vi "VIH HelpGen - Image - Fill Outer Regions in 2D Array.vi"(8 "New Color (transparent)":u32(colorbox)=16777216, 9 "Source Color (white)":u32=16777215 format="%.0x", 11 "Image Data in":u32[][](array[numeric]) format="%.0x") -> (3 "Image Data out":u32[][](array[numeric]) format="%.0x")   [LabVIEW 2014]
doc: "::: VI Helpeks :::\nCopyright (c) 2000-2026 Konstantin Shifershteyn. All rights reserved."
panel:
  out "Points replaces":i32
  out "Sub-regions found":i32
  # "VI Helpeks\nCopyright (c) 2012-2026 Konstantin Shifershteyn"
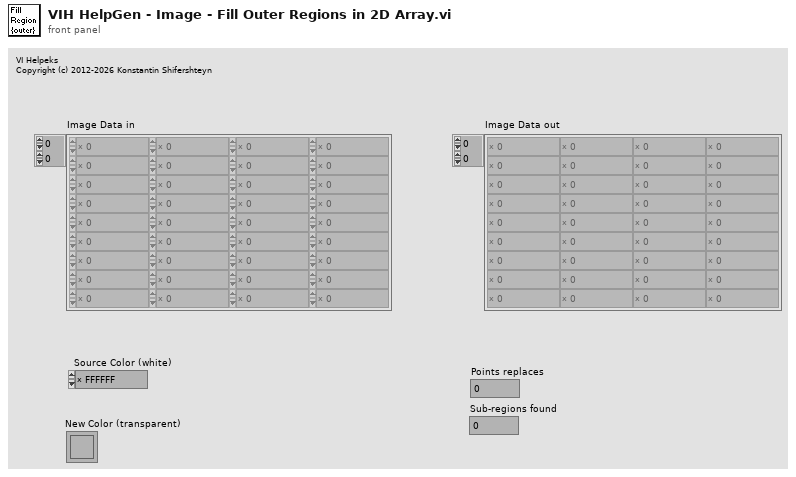
[diagram p1: front panel]
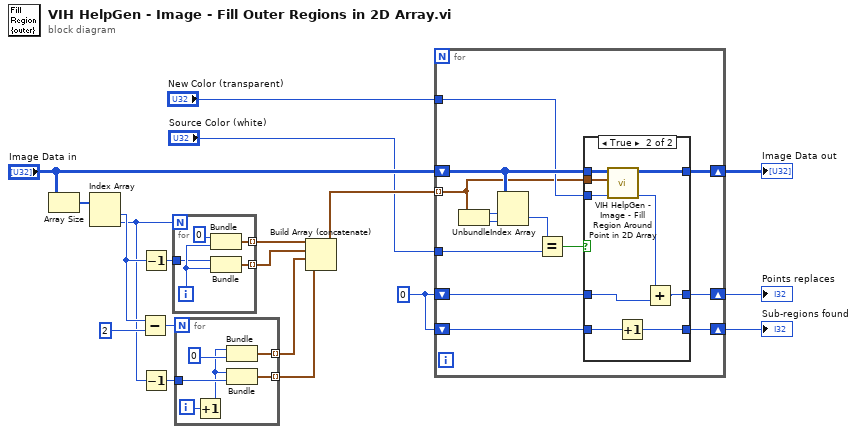
[diagram p0: block diagram]
diagram:
  w2 = 0
  n1 = Array Size(array="Image Data in") -> (size(s)=w19:i32[])
  n2 = Index Array(array=w19) -> (element #1=w10:i32, element #2=w9:i32)  [unwired: 2 in]
  n3 = Subtract(x=w10, y=2) -> (x-y=w11:i32)
  n4 = Decrement(x=w10) -> (x-1=w18:i32)
  n5 = Decrement(x=w9) -> (x-1=w15:i32)
  n6 = for {
    N: w9 -> [_]
    tunnel: w18 -> [w23]
    tunnel: [w21] -> w17 mode=indexing
    tunnel: [w20] -> w16 mode=indexing
    i -> [w24]
    n7 = Bundle(0, w24) -> (w21:cluster{i32, i32})  [unwired: 1 in]
    n8 = Bundle(w23, w24) -> (w20:cluster{i32, i32})  [unwired: 1 in]
  }
  n9 = for {
    N: w11 -> [_]
    tunnel: [w30] -> w13 mode=indexing
    tunnel: [w29] -> w12 mode=indexing
    tunnel: w15 -> [w28]
    i -> [w26]
    n10 = Increment(x=w26) -> (x+1=w25:i32)
    n11 = Bundle(w25, 0) -> (w30:cluster{i32, i32})  [unwired: 1 in]
    n12 = Bundle(w25, w28) -> (w29:cluster{i32, i32})  [unwired: 1 in]
  }
  n13 = Build Array (concatenate)(w17, w16, w13, w12) -> (w7:cluster{i32, i32}[])
  n14 = for {
    shift-right: [w38] -> w4
    shift-left: "Image Data in" -> [w39]
    tunnel: w7 -> [w31] mode=indexing
    tunnel: "Source Color (white)" -> [w40]
    tunnel: "New Color (transparent)" -> [w36]
    shift-right: [w34] -> w3
    shift-left: w2 -> [w35]
    shift-right: [w32] -> w1
    shift-left: w2 -> [w33]
    n15 = Unbundle(w31) -> (w43:i32, w42:i32)
    n16 = Index Array(array=w39, index (row)=w43, index (col)=w42) -> (element=w41:u32)
    n17 = Equal?(x=w41, y=w40) -> (x = y?=w37:bool)
    n18 = case shown="True" w37 {
      tunnel: w39 -> [w46 w55]
      tunnel: [w46 w54] -> w38
      tunnel: w36 -> [_ w53]
      tunnel: w35 -> [w45 w52]
      tunnel: [w45 w51] -> w34
      tunnel: w33 -> [w44 w49]
      tunnel: [w44 w48] -> w32
      tunnel: w31 -> [_ w47]
      frame False {
      }
      frame True {
        n19 = call "VIH HelpGen - Image - Fill Region Around Point in 2D Array.vi"("New Color (transparent)"=w53, "Point coords (0,0)"=w47, "Image Data in"=w55) -> ("Replacements"=w50:i32, "Image Data out"=w54:u32[][])  [unwired: 7 in]
        n20 = Increment(x=w49) -> (x+1=w48:i32)
        n21 = Add(x=w50, y=w52) -> (x+y=w51:i32)
      }
    }
  }
  "Image Data out" <- w4
  "Sub-regions found" <- w1
  "Points replaces" <- w3
